vi "Lidar_Machine_etats.vi"() -> ()   [LabVIEW 2017]
uses:
  enum_etats_lidar.ctl
  <vilib>/Platform/TimedLoop/XDataNode/timing_clust.ctl
  <vilib>/Platform/TimedLoop/XDataNode/nitl_modes.ctl
  <vilib>/Platform/TimedLoop/XDataNode/wakeup.ctl
  enum_zone.ctl
  <vilib>/platform/TimedLoop/XDataNode/XDataNode.xnode
  <vilib>/Platform/TimedLoop/XDataNode/XDNodeRunTimeDep.lvlib
panel:
  out "Espace libre":dbl[][](array[numeric])
  out "Zone 3":dbl[][](array[numeric])
  out "Zone 2":dbl[][](array[numeric])
  out "Timeout":bool=TRUE
  out "Selection de état":T1
  in  "stop":bool
  out "Tableau lidar":dbl[][](array[numeric])=[[0.0, 1.0, 2.0, 3.0, 4.0, 5.0, 6.0, 7.0, 8.0, 9.0, 10.0, 11.0, 12.0, 13.0, 14.0, 15.0, 16.0, 17.0, 18.0, 19.0, 20.0, 21.0, 22.0, 23.0, 24.0, 25.0, 26.0, 27.0, 28.0, 29.0, 30.0, 31.0, 32.0, 33.0, 34.0, 35.0], [20.0, 15.0, 30.0, 31.0, 42.0, 50.0, 51.0, 60.0, 20.0, 15.0, 30.0, 31.0, 42.0, 50.0, 51.0, 60.0, 20.0, 15.0, 30.0, 31.0, 42.0, 50.0, 51.0, 60.0, 20.0, 15.0, 30.0, 31.0, 42.0, 50.0, 51.0, 60.0, 20.0, 15.0, 30.0, 31.0], [0.0, 0.0, 0.0, 0.0, 0.0, 0.0, 0.0, 0.0, 0.0, 0.0, 0.0, 0.0, 0.0, 0.0, 0.0, 0.0, 0.0, 0.0, 0.0, 0.0, 0.0, 0.0, 0.0, 0.0, 0.0, 0.0, 0.0, 0.0, 0.0, 0.0, 0.0, 0.0, 0.0, 0.0, 0.0, 0.0]]
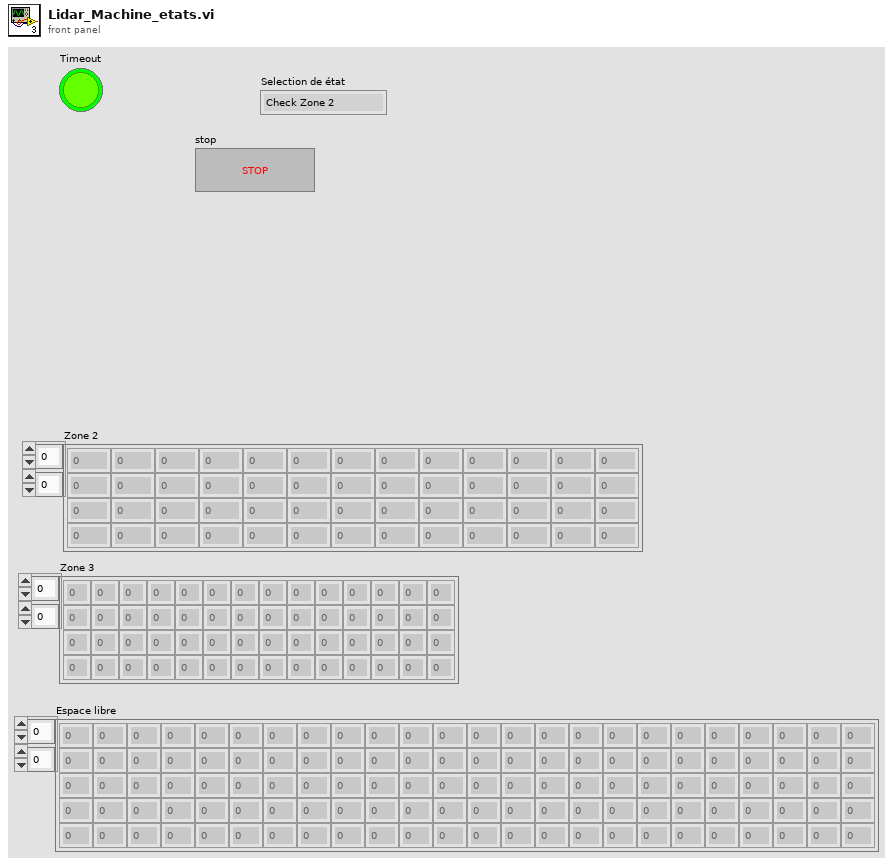
[diagram p1: front panel]
types:
  T1 = typedef "enum_etats_lidar.ctl" = enum16{"Check Zone 2", "Obstacle Zone 2", "Check Zone 3", "Obstacle Zone 3", "Avance", "Obstacle Timer", "Rescan 10s", "Check Zone 3 Bis", "Rotation new direction", "Rotation 180", "Timeout ?", "Arret complet", "Rotation new dir timer", "Rotation 180 timer"}
  T2 = typedef "enum_zone.ctl" = enum16{"Zone_2", "Zone_3", "Espace_libre", "Aucune"}
  T3 = typedef "XDNodeRunTimeDep.lvlib/timing_clust.ctl" = cluster{"Expected End [f-1]":u64, "Actual End [f-1]":u64, "Finished Late? [f-1]":bool, "Expected End [i-1]":u64, "Actual End [i-1]":u64, "Finished Late? [i-1]":bool, "Expected Start [i]":u64, "Actual Start [i]":u64, "Expected Start [f]":u64, "Actual Start [f]":u64, "Source Name":string, "Structure Name":string, "Period":i64, "Deadline":i64, "Offset":i64, "Start":i64, "Priority":i32, "Timeout":i32, "Mode":T4, "Wakeup Reason":T5, "Error":errorcluster, "Source Type":string, "Secondary Source Type":string, "Global End Time":u64, "Global Start Time":u64, "Frame Duration":u64, "Iteration Duration":u64, "Assigned CPU":i32, "I/O Scan Engine Mode":u32}
  T4 = typedef "XDNodeRunTimeDep.lvlib/nitl_modes.ctl" = enum32{"No Change", "Process missed periods, maintain original phase", "Discard missed periods, maintain original phase", "Process missed periods, ignore original phase", "Discard missed periods, ignore original phase"}
  T5 = typedef "XDNodeRunTimeDep.lvlib/wakeup.ctl" = enum32{"Normal", "Aborted", "Asynchronous wakeup", "Timing source error", "Timed loop error", "Timeout"}
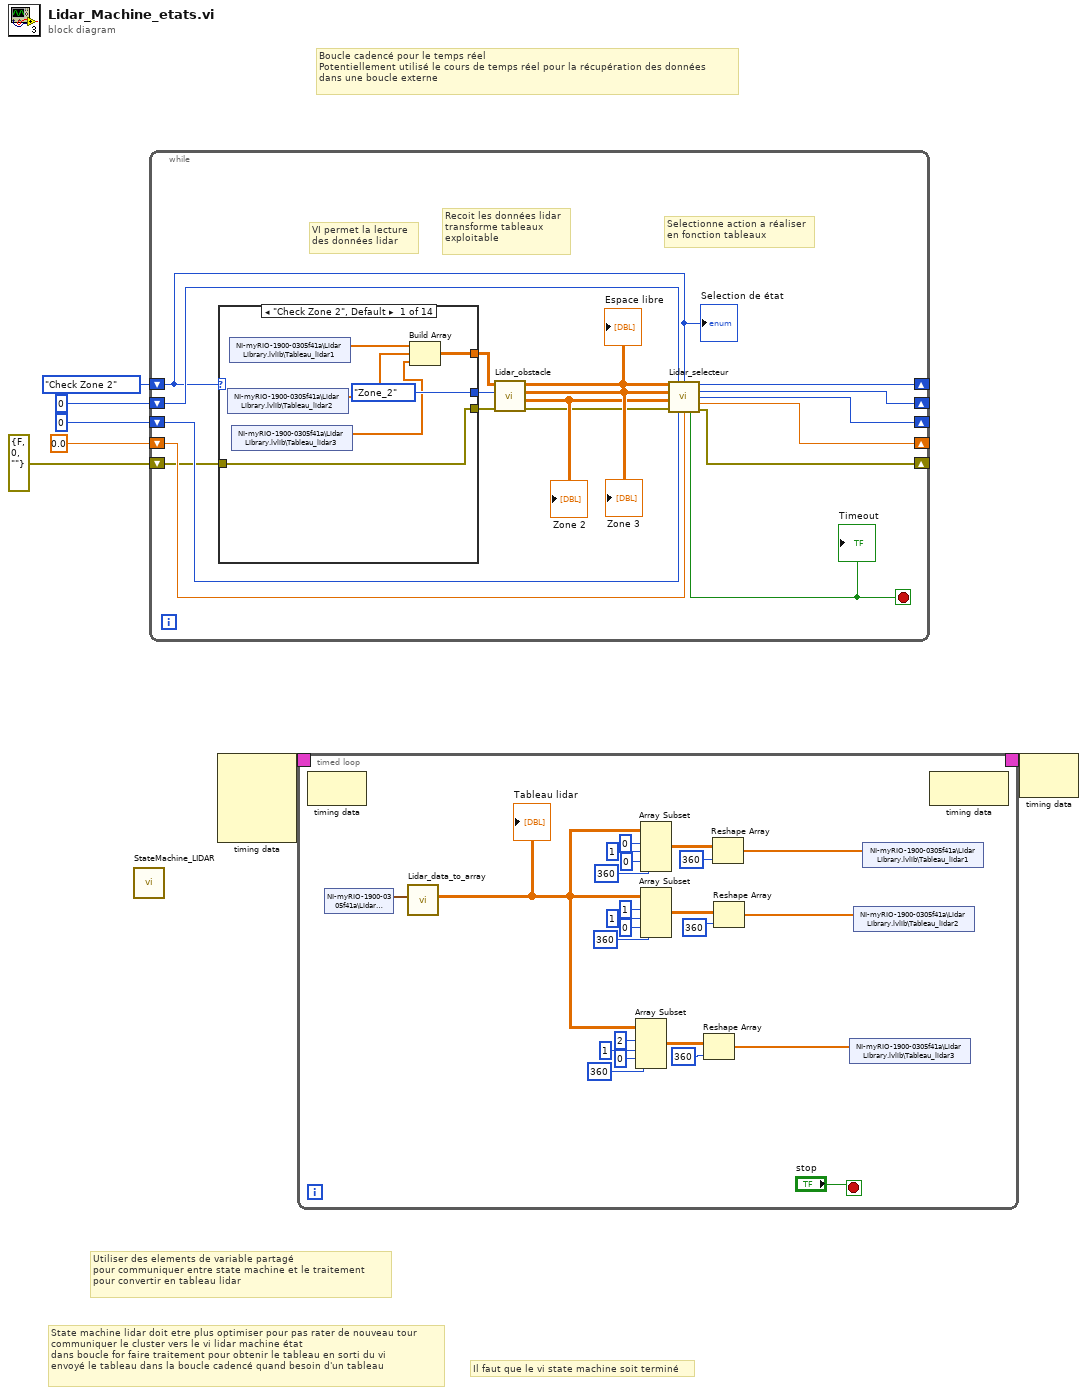
[diagram p0: block diagram]
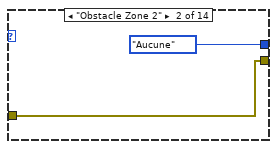
[diagram p2: hidden frame]
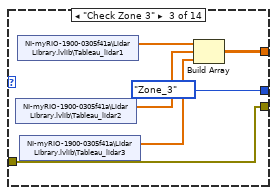
[diagram p3: hidden frame]
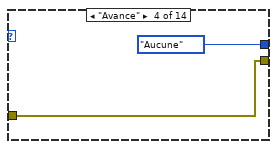
[diagram p4: hidden frame]
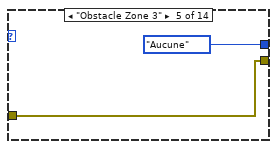
[diagram p5: hidden frame]
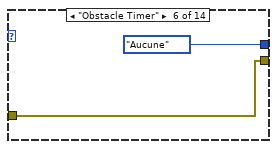
[diagram p6: hidden frame]
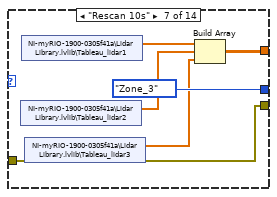
[diagram p7: hidden frame]
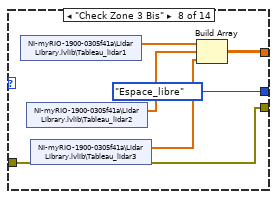
[diagram p8: hidden frame]
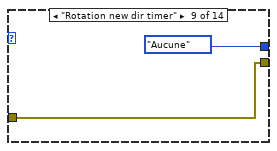
[diagram p9: hidden frame]
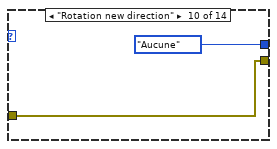
[diagram p10: hidden frame]
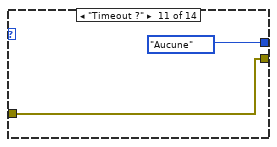
[diagram p11: hidden frame]
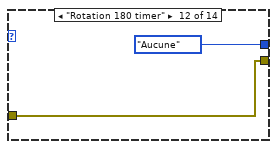
[diagram p12: hidden frame]
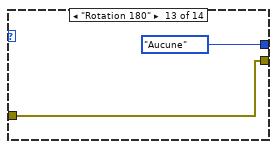
[diagram p13: hidden frame]
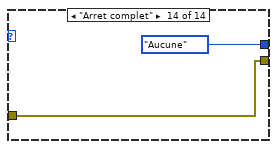
[diagram p14: hidden frame]
diagram:
  # "State machine lidar doit etre plus optimiser pour pas rater de nouveau tour\ncommuniquer le cluster vers le vi lidar machine état\ndans boucle for faire traitement pour obtenir le tableau en sorti du vi\nenvoyé le tableau dans la boucle cadencé quand besoin d'un tableau"
  # "Utiliser des elements de variable partagé\npour communiquer entre state machine et le traitement \npour convertir en tableau lidar"
  # "Il faut que le vi state machine soit terminé"
  # "Boucle cadencé pour le temps réel\nPotentiellement utilisé le cours de temps réel pour la récupération des données \ndans une boucle externe"
  n1 = call "StateMachine_LIDAR.vi"() -> ()  [unwired: 12 in]
  n2 = while {
    shift-right: [w21] -> _
    shift-left: enum_etats_lidar."Check Zone 2" ("Selection de état") -> [w12]
    shift-right: [w19] -> _
    shift-left: u32 0 ("Timeout Count") -> [w20]
    shift-right: [w18] -> _
    shift-left: u32 0 ("Tick Count(mSec)") -> [w17]
    shift-right: [w15] -> _
    shift-left: 0.0 ("New Angle") -> [w16]
    shift-right: [w13] -> _
    shift-left: errorcluster {"status"=FALSE, "code"=0, "source"=""} ("error out") -> [w10]
    stop <- w14 stop-if-true
    # "VI permet la lecture \ndes données lidar"
    # "Selectionne action a réaliser\nen fonction tableaux"
    # "Recoit les données lidar\ntransforme tableaux \nexploitable"
    n3 = case shown="\"Check Zone 2\", Default" w12 {
      tunnel: [enum_zone."Zone_2" ("Enum Zone") enum_zone."Aucune" ("Enum Zone") enum_zone."Zone_3" ("Enum Zone") enum_zone."Aucune" ("Enum Zone") enum_zone."Aucune" ("Enum Zone") enum_zone."Aucune" ("Enum Zone") enum_zone."Zone_3" ("Enum Zone") enum_zone."Espace_libre" ("Enum Zone") enum_zone."Aucune" ("Enum Zone") enum_zone."Aucune" ("Enum Zone") enum_zone."Aucune" ("Enum Zone") enum_zone."Aucune" ("Enum Zone") enum_zone."Aucune" ("Enum Zone") enum_zone."Aucune" ("Enum Zone")] -> w11
      tunnel: w10 -> [w30 w32 w38 w40 w42 w44 w50 w56 w58 w60 w62 w64 w66 w68]
      tunnel: [w30 w32 w38 w40 w42 w44 w50 w56 w58 w60 w62 w64 w66 w68] -> w9
      tunnel: [w26 _ w34 _ _ _ w49 w55 _ _ _ _ _ _] -> w8
      frame "Check Zone 2", Default {
        n4 = shared-variable "NI-myRIO-1900-0305f41a\\Lidar Library.lvlib\\Tableau_lidar2"() -> (w28:dbl[])  [unwired: 1 in, 1 out]
        n5 = shared-variable "NI-myRIO-1900-0305f41a\\Lidar Library.lvlib\\Tableau_lidar1"() -> (w29:dbl[])  [unwired: 1 in, 1 out]
        n6 = shared-variable "NI-myRIO-1900-0305f41a\\Lidar Library.lvlib\\Tableau_lidar3"() -> (w27:dbl[])  [unwired: 1 in, 1 out]
        n7 = Build Array(w29, w28, w27) -> (w26:dbl[][])
      }
      frame "Obstacle Zone 2" {
      }
      frame "Check Zone 3" {
        n8 = shared-variable "NI-myRIO-1900-0305f41a\\Lidar Library.lvlib\\Tableau_lidar2"() -> (w36:dbl[])  [unwired: 1 in, 1 out]
        n9 = shared-variable "NI-myRIO-1900-0305f41a\\Lidar Library.lvlib\\Tableau_lidar1"() -> (w37:dbl[])  [unwired: 1 in, 1 out]
        n10 = shared-variable "NI-myRIO-1900-0305f41a\\Lidar Library.lvlib\\Tableau_lidar3"() -> (w35:dbl[])  [unwired: 1 in, 1 out]
        n11 = Build Array(w37, w36, w35) -> (w34:dbl[][])
      }
      frame "Avance" {
      }
      frame "Obstacle Zone 3" {
      }
      frame "Obstacle Timer" {
      }
      frame "Rescan 10s" {
        n12 = shared-variable "NI-myRIO-1900-0305f41a\\Lidar Library.lvlib\\Tableau_lidar2"() -> (w47:dbl[])  [unwired: 1 in, 1 out]
        n13 = shared-variable "NI-myRIO-1900-0305f41a\\Lidar Library.lvlib\\Tableau_lidar1"() -> (w48:dbl[])  [unwired: 1 in, 1 out]
        n14 = shared-variable "NI-myRIO-1900-0305f41a\\Lidar Library.lvlib\\Tableau_lidar3"() -> (w46:dbl[])  [unwired: 1 in, 1 out]
        n15 = Build Array(w48, w47, w46) -> (w49:dbl[][])
      }
      frame "Check Zone 3 Bis" {
        n16 = shared-variable "NI-myRIO-1900-0305f41a\\Lidar Library.lvlib\\Tableau_lidar1"() -> (w54:dbl[])  [unwired: 1 in, 1 out]
        n17 = shared-variable "NI-myRIO-1900-0305f41a\\Lidar Library.lvlib\\Tableau_lidar2"() -> (w53:dbl[])  [unwired: 1 in, 1 out]
        n18 = shared-variable "NI-myRIO-1900-0305f41a\\Lidar Library.lvlib\\Tableau_lidar3"() -> (w52:dbl[])  [unwired: 1 in, 1 out]
        n19 = Build Array(w54, w53, w52) -> (w55:dbl[][])
      }
      frame "Rotation new dir timer" {
      }
      frame "Rotation new direction" {
      }
      frame "Timeout ?" {
      }
      frame "Rotation 180 timer" {
      }
      frame "Rotation 180" {
      }
      frame "Arret complet" {
      }
    }
    n20 = call "Lidar_obstacle.vi"("error in (no error)"=w9, "Enum Zone"=w11, "Tableau lidar"=w8) -> ("error out"=w22:errorcluster, "Zone 2"=w23:dbl[][], "Zone 3"=w24:dbl[][], "Espace libre"=w25:dbl[][])  [unwired: 5 in]
    "Zone 2" <- w23
    "Zone 3" <- w24
    "Espace libre" <- w25
    n21 = call "Lidar_selecteur.vi"("Espace dispo"=w25, "Timeout Count"=w20, "Enum état"=w12, "Zone 3"=w24, "Zone 2"=w23, "error in (no error)"=w22, "Tick Count(mSec)"=w17, "New Angle"=w16) -> ("Selection de état"=w21:T1, "Timeout Count"=w19:u32, "Tick Count(mSec)"=w18:u32, "New Angle"=w15:dbl, "Timeout"=w14:bool, "error out"=w13:errorcluster)  [unwired: 2 in]
    "Timeout" <- w14
    "Selection de état" <- w12
  }
  n22 = node-c288() -> (w2:T3)  [unwired: 4 in]
  n23 = timed-loop {
    timing: w2 -> [_]
    timing-out: [_] -> w1
    stop <- "stop" stop-if-true
    n24 = node-c288() -> ()  [unwired: 1 in, 1 out]
    n25 = shared-variable "NI-myRIO-1900-0305f41a\\Lidar Library.lvlib\\Data"() -> (w92:cluster{"Angle":dbl, dbl}[])  [unwired: 1 in, 1 out]
    n26 = call "Lidar_data_to_array.vi"("Data"=w92) -> ("Tableau lidar"=w91:dbl[][])  [unwired: 10 in]
    "Tableau lidar" <- w91
    n27 = Array Subset(array=w91, index (row)=2 ("index"), length (row)=1 ("length"), index (col)=0 ("index"), length (col)=360 ("length")) -> (w74:dbl[][])
    n28 = Array Subset(array=w91, index (row)=0 ("index"), length (row)=1 ("length"), index (col)=0 ("index"), length (col)=360 ("length")) -> (w78:dbl[][])
    n29 = Array Subset(array=w91, index (row)=1 ("index"), length (row)=1 ("length"), index (col)=0 ("index"), length (col)=360 ("length")) -> (w73:dbl[][])
    n30 = Reshape Array(w74, 360 ("dimension size")) -> (w70:dbl[])
    n31 = Reshape Array(w78, 360 ("dimension size")) -> (w72:dbl[])
    n32 = Reshape Array(w73, 360 ("dimension size")) -> (w71:dbl[])
    n33 = shared-variable "NI-myRIO-1900-0305f41a\\Lidar Library.lvlib\\Tableau_lidar3"(w70) -> ()  [unwired: 1 in, 1 out]
    n34 = shared-variable "NI-myRIO-1900-0305f41a\\Lidar Library.lvlib\\Tableau_lidar2"(w71) -> ()  [unwired: 1 in, 1 out]
    n35 = shared-variable "NI-myRIO-1900-0305f41a\\Lidar Library.lvlib\\Tableau_lidar1"(w72) -> ()  [unwired: 1 in, 1 out]
    n36 = node-c288() -> ()  [unwired: 1 in, 1 out]
  }
  n37 = node-c288(w1) -> ()  [unwired: 1 out]
